vi "TCP Server Get Instance Semaphore RefNum.vi"(8 "error out":errorcluster, 11 "RefNum":refnum<class "JKI TCP Server.lvclass">) -> (0 "error in (no error)":errorcluster, 2 "semaphore":T1, 3 "dup RefNum":refnum<class "JKI TCP Server.lvclass">)   [LabVIEW 2020, in "JKI TCP Server.lvclass"]
uses:
  JKI TCP Server.lvclass
  JKI TCP Server.lvclass/JKI TCP Server.ctl
panel:
  # "<VI NAME>\n\n<DESCRIPTION>\n\nCopyright (C) 2003 Jim Kring jim@jimkring.com\n\nPlease visit http://www.OpenG.org to learn about the\nOpen Source LabVIEW software movement.\n\nThis library is free software; you can redistribute it and/or\nmodify it under the terms of the GNU Lesser General Public\nLicense as published by the Free Software Foundation; either\nversion 2.1 of the License, or (at your option) any later version.\nThis library is distributed in the hope that it will be useful,\nbut WITHOUT ANY WARRANTY; without even the implied warranty of\nMERCHANTABILITY or FITNESS FOR A PARTICULAR PURPOSE. See the GNU\nLesser General Public License for more details.\nYou should have received a copy of the GNU Lesser General Public\nLicense along with this library; if not, write to the Free Software\nFoundation, Inc., 59 Temple Place, Suite 330, Boston, MA 02111-1307 USA"
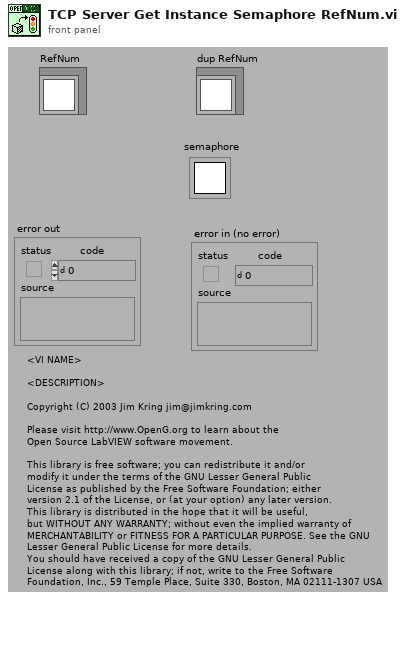
[diagram p1: front panel]
types:
  T1 = typedef "Semaphore RefNum" = refnum<k1>
  T2 = typedef "JKI TCP Server.lvclass/TCP Server Object RefNum.ctl" = refnum<k1>
  T3 = typedef "JKI TCP Server.lvclass/TCP Server Object RefNum - Enum.ctl" = enum16{"TCP Server"}
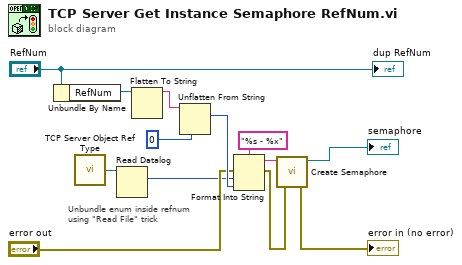
[diagram p0: block diagram]
diagram:
  # "Unbundle enum inside refnum using \"Read File\" trick"
  n1 = Unbundle By Name("RefNum") -> ("RefNum"=w1:T2)
  n2 = call "TCP Server Object Ref Type.vi"() -> ("Object RefNum Type"=w4:T2)  [unwired: 5 in]
  n3 = Read Datalog(7:w4) -> (2:w3:T3)  [unwired: 2 in, 2 out]
  n4 = Flatten To String(anything=w1) -> (data string=w13:string)  [unwired: 3 in, 2 out]
  n5 = Unflatten From String(type=u32 0 ("input 2"), binary string=w13) -> (value=w12:u32)  [unwired: 3 in, 2 out]
  n6 = Format Into String(format string="%s - %x", error in="error out", w3, w12) -> (resulting string=w9:string, error out=w10:errorcluster)  [unwired: 1 in]
  n7 = call <vilib>:"Create Semaphore.vi"("error in (no error)"=w10, "name (unnamed)"=w9) -> ("error out"=→"error in (no error)":errorcluster, "semaphore"=→"semaphore":T1)  [unwired: 3 in, 1 out]
  "dup RefNum" <- "RefNum"
